vi "Open Template.vi"(8 "error in":errorcluster, 10 "Template":path, 11 "ILabVIEWFile in":refnum<class "ILabVIEW File.lvclass">) -> (0 "error out":errorcluster, 3 "ILabVIEWFile out":refnum<class "ILabVIEW File.lvclass">)   [LabVIEW 2026, in "ILabVIEW File.lvclass"]
doc: "Open template (specified by file) and store reference in the class private data."
uses:
  ILabVIEW File.lvclass
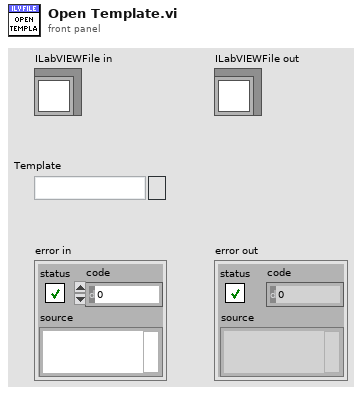
[diagram p1: front panel]
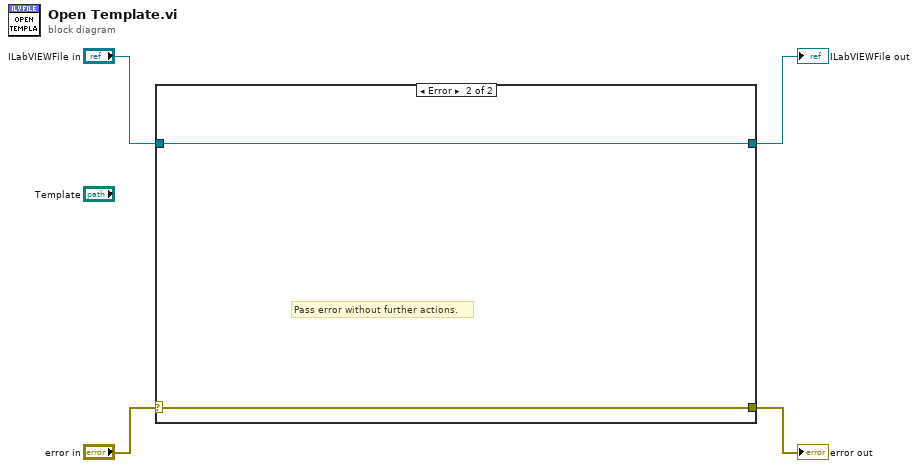
[diagram p0: block diagram]
diagram:
  n1 = case shown="Error" "error in" {
    selector: "error in" -> [w6 w8]
    tunnel: [w6 w8] -> w3
    tunnel: [w5 w7] -> w1
    tunnel: "ILabVIEWFile in" -> [w5 w7]
    frame No Error {
    }
    frame Error {
      # "Pass error without further actions."
    }
  }
  "error out" <- w3
  "ILabVIEWFile out" <- w1
